vi "[ce] Limit.vi"(5 "delta":dbl=1e-10 format="%.2e", 6 "error in":errorcluster, 7 "formula info":cluster{"formula":string, "x-variable":string}, 9 "point":dbl format="%.2f") -> (0 "error out":errorcluster, 1 "ticks":u32, 2 "right limit":dbl format="%.8e", 3 "left limit":dbl format="%.8e")   [LabVIEW 2021]
doc: "Determines the left and right limits of a 1D function at the given point.\n\n::: CalcExpress Toolkit :::\nCopyright (c) 2000-2026 Konstantin Shifershteyn. All rights reserved."
panel:
  # "Example:\n\n point: 0.0\n delta: 1.0E-10\n formula info:\n    formula:    sin(t)/t \n    x-variable: t"
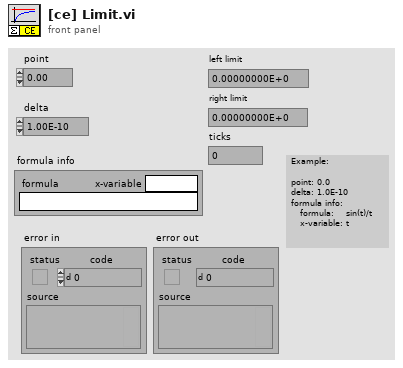
[diagram p1: front panel]
types:
  T1 = enum16{"create", "destroy", "set value", "get value"}
  T2 = typedef "VarMan Variable Context Handle.ctl" = i32
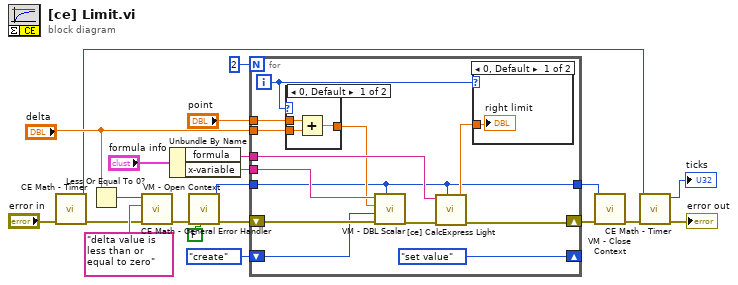
[diagram p0: block diagram]
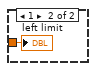
[diagram p2: hidden frame]
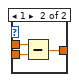
[diagram p3: hidden frame]
diagram:
  n1 = call "CE Math - Timer.vi"("error in (no error)"="error in") -> ("error out"=w9:errorcluster, "ticks out"=w2:u32)  [unwired: 7 in]
  n2 = Less Or Equal To 0?(x="delta") -> (x <= 0?=w21:bool)
  n3 = call "CE Math - General Error Handler.vi"("error before"=w9, "message"="delta value is less than or equal to zero", "error? (T)"=w21) -> ("error out"=w19:errorcluster)  [unwired: 5 in, 1 out]
  n4 = Unbundle By Name("formula info") -> ("formula"=w15:string, "x-variable"=w14:string)
  n5 = call "VM - Open Context.vi"("close loose contexts (F)"=FALSE ("close loose contexts (T)"), "error in"=w19) -> ("error out"=w18:errorcluster, "VC Handle out"=w16:T2)  [unwired: 7 in, 1 out]
  n6 = for {
    N: 2 -> [_]
    shift-right: [w28] -> w7
    shift-left: w18 -> [w34]
    shift-right: [T1."set value" ("cmd")] -> _
    shift-left: T1."create" ("cmd") -> [w33]
    tunnel: w16 -> [w22]
    tunnel: w15 -> [w29]
    tunnel: w14 -> [w30]
    tunnel: "point" -> [w25]
    tunnel: "delta" -> [w24]
    tunnel: [w22] -> w5
    i -> [w27]
    n7 = case shown="0, Default" w27 {
      tunnel: w25 -> [w39 w42]
      tunnel: w24 -> [w38 w41]
      tunnel: [w37 w40] -> w23
      frame 0, Default {
        n8 = Add(x=w39, y=w38) -> (x+y=w37:dbl)
      }
      frame 1 {
        n9 = Subtract(x=w42, y=w41) -> (x-y=w40:dbl)
      }
    }
    n10 = call "VM - DBL Scalar.vi"("VC Handle"=w22, "error in"=w34, "cmd"=w33, "value in"=w23, "name_spec"=w30) -> ("error out"=w31:errorcluster)  [unwired: 1 in, 5 out]
    n11 = call "[ce] CalcExpress Light.vi"("VC Handle"=w22, "error in"=w31, "expression"=w29) -> ("error out"=w28:errorcluster, "numeric value"=w26:dbl)  [unwired: 6 in, 1 out]
    n12 = case shown="0, Default" w27 {
      tunnel: w26 -> [w35 w36]
      frame 0, Default {
        "right limit" <- w35
      }
      frame 1 {
        "left limit" <- w36
      }
    }
  }
  n13 = call "VM - Close Context.vi"("error in"=w7, "VC Handle"=w5) -> ("error out"=w6:errorcluster)  [unwired: 8 in, 1 out]
  n14 = call "CE Math - Timer.vi"("error in (no error)"=w6, "ticks in"=w2) -> ("error out"=→"error out":errorcluster, "ticks out"=→"ticks":u32)  [unwired: 6 in]
